vi "Close.vi"(8 "error in (no error)":errorcluster, 11 "PGJDPResult in":refnum<class "Result.lvclass">) -> (0 "error out":errorcluster)   [LabVIEW 2020, in "ORM_pgsql_jdp.lvlib" / "Result.lvclass"]
uses:
  Result.lvclass
  Result.lvclass/Result.ctl
  <vilib>/JDP Science/PostgreSQL Library/Result/PQ Result.lvclass
  <vilib>/Viviota/shared/ORM.lvlibp/Query Result/Query Result.lvclass
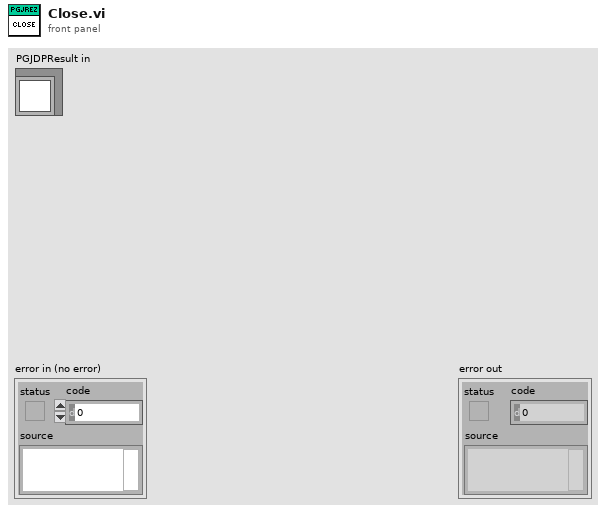
[diagram p1: front panel]
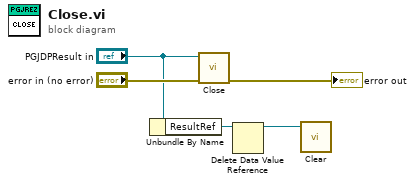
[diagram p0: block diagram]
diagram:
  n1 = Unbundle By Name("PGJDPResult in") -> ("ResultRef"=w2:refnum<data-value>)
  n2 = call-parent "Close.vi"("error in (no error)"="error in (no error)", "Query Result in"="PGJDPResult in") -> ("error out"=→"error out":errorcluster)  [unwired: 9 in]
  n3 = Delete Data Value Reference(data value reference=w2) -> (data value=w1:refnum<class "PQ Result.lvclass">)  [unwired: 1 in, 1 out]
  n4 = call <vilib>:"Clear.vi"("PQ Result  in"=w1) -> ()  [unwired: 10 in, 1 out]
